vi "write maintance.vi"(9 "data":variant, 10 "station":string, 11 "URL":string) -> (3 "ok?":bool)   [LabVIEW 2012]
uses:
  write_bool.vi
  Globals/Global.vi
  read_Array.vi
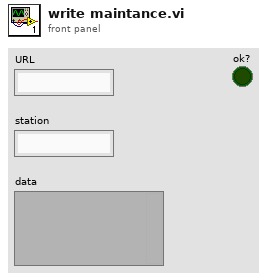
[diagram p1: front panel]
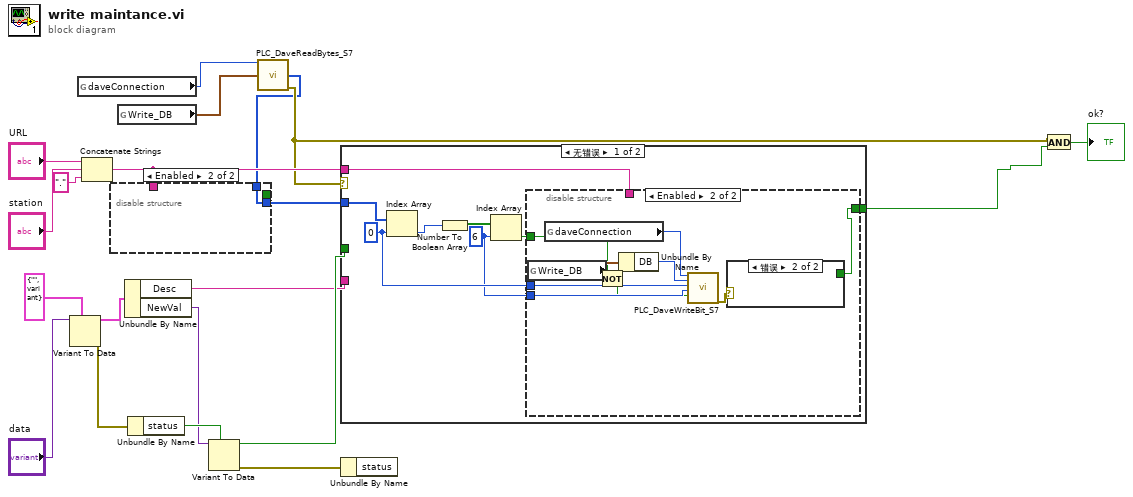
[diagram p0: block diagram]
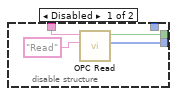
[diagram p2: hidden frame]
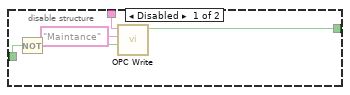
[diagram p3: hidden frame]
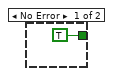
[diagram p4: hidden frame]
diagram:
  n1 = Variant To Data(type=cluster{"Desc":string, "NewVal":variant} {"Desc"="", "NewVal"=variant} ("output cluster"), Variant="data") -> (data=w14:cluster{"Desc":string, "NewVal":variant}, error out=w12:errorcluster)  [unwired: 1 in]
  n2 = global read "Global.vi" "daveConnection"() -> (w3:i64)
  n3 = Concatenate Strings("URL", "station", "." ("string")) -> (w7:string)
  n4 = global read "Global.vi" "Write_DB"() -> (w4:cluster{"DB":i32, "start":i32, "len":i32})
  n5 = Unbundle By Name(w14) -> ("Desc"=w15:string, "NewVal"=w16:variant)
  n6 = Unbundle By Name(w12) -> ("status"=w17:bool)
  n7 = Variant To Data(type=w17, Variant=w16) -> (data=w19:bool, error out=w18:errorcluster)  [unwired: 1 in]
  n8 = call "PLC_DaveReadBytes_S7.vi"("daveConnection in"=w3, "地址"=w4) -> ("read Buffer"=w1:u8[], "error out"=w2:errorcluster)  [unwired: 10 in, 2 out]
  n9 = disable-structure shown="Enabled" {
    disable-tunnel: [w24 w25] -> w10
    disable-tunnel: w7 -> [w23 _]
    disable-tunnel: [w21 _] -> _
    disable-tunnel: w1 -> [_ w25]
    frame Disabled {
      n10 = call-poly "OPC Read.vi"("Address"="Read", "URL"=w23) -> ("Value"=w24:u8[], "ok?"=w21:bool)  [unwired: 7 in, 1 out]
    }
    frame Enabled {
    }
  }
  n11 = case shown="无错误" w2 {
    tunnel: w7 -> [w29 _]
    tunnel: w10 -> [w33 _]
    tunnel: w19 -> [_ _]
    tunnel: w15 -> [_ _]
    tunnel: [w28 _] -> w5
    frame No Error {
      w26 = 6 ("index")
      w27 = 0 ("index")
      n12 = Index Array(array=w33, index=w27) -> (element=w32:u8)
      n13 = Number To Boolean Array(number=w32) -> (Boolean array=w31:bool[])
      n14 = Index Array(array=w31, index=w26) -> (element=w30:bool)
      n15 = disable-structure shown="Enabled" {
        disable-tunnel: w30 -> [w38 w42]
        disable-tunnel: w29 -> [w37 _]
        disable-tunnel: [w34 w39] -> w28
        disable-tunnel: w27 -> [_ w44]
        disable-tunnel: w26 -> [_ w43]
        frame Disabled {
          n16 = Not(x=w38) -> (.not. x?=w35:bool)
          n17 = call-poly "OPC Write.vi"("Value"=w35, "Address"="Maintance", "URL"=w37) -> ("ok?"=w34:bool)  [unwired: 7 in, 1 out]
        }
        frame Enabled {
          n18 = global read "Global.vi" "Write_DB"() -> (w45:cluster{"DB":i32, "start":i32, "len":i32})
          n19 = global read "Global.vi" "daveConnection"() -> (w46:i64)
          n20 = Not(x=w42) -> (.not. x?=w41:bool)
          n21 = Unbundle By Name(w45) -> ("DB"=w47:i32)
          n22 = call "PLC_DaveWriteBit_S7.vi"("daveConnection IN"=w46, "DB"=w47, "byte"=w44, "bit"=w43, "value"=w41) -> ("error out"=w40:errorcluster)  [unwired: 12 in, 2 out]
          n23 = case shown="错误" w40 {
            tunnel: [TRUE ("ok?") _] -> w39
            frame No Error {
            }
            frame Error {
            }
          }
        }
      }
    }
    frame Error {
    }
  }
  n24 = Unbundle By Name(w18) -> ()  [unwired: 1 out]
  n25 = And(x=w2, y=w5) -> (x .and. y?=→"ok?":bool)
